vi "convertToHtml.vi"(8 "error in (no error)":errorcluster, 10 "HTML File Path":path, 11 "MS-Excel in":refnum<class "MS-Excel.lvclass">) -> (0 "error out":errorcluster, 3 "MS-Excel out":refnum<class "MS-Excel.lvclass">)   [LabVIEW 2017, in "LabVIEW NPOI.lvlib" / "MS-Excel.lvclass"]
uses:
  MS-Excel.lvclass
  MS-Excel.lvclass/MS-Excel.ctl
  C:/Program Files (x86)/National Instruments/LabVIEW 2017/vi.lib/BenjaminR/LabVIEW NPOI/lib/NPOI 2.1.1/NPOI.OOXML.dll
  Program Files (x86)/National Instruments/LabVIEW 2017/vi.lib/BenjaminR/LabVIEW NPOI/lib/NPOI 2.1.1/NPOI.OOXML.dll
  System.Xml
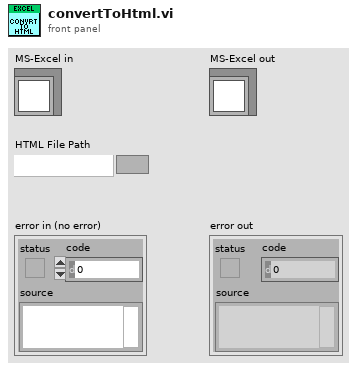
[diagram p1: front panel]
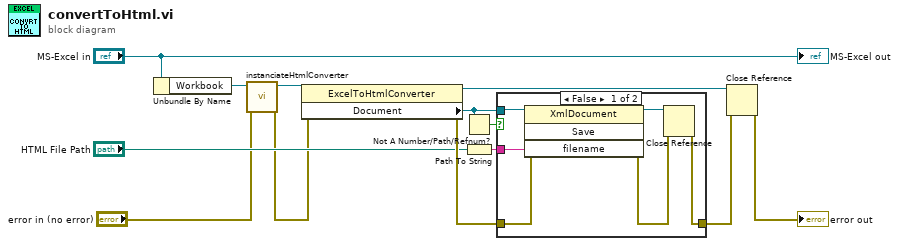
[diagram p0: block diagram]
diagram:
  n1 = Unbundle By Name("MS-Excel in") -> ("Workbook"=w3:refnum<k24>)
  n2 = call "instanciateHtmlConverter.vi"("error in (no error)"="error in (no error)", "workbook"=w3) -> ("error out"=w1:errorcluster, "ExcelToHtmlConverter"=w4:refnum<k24>)  [unwired: 8 in]
  n3 = property class="ExcelToHtmlConverter"(reference=w4, error in=w1) -> (reference out=w10:refnum<k24>, error out=w12:errorcluster, "Document"=w6:refnum<k24>)
  n4 = Not A Number/Path/Refnum?(number/path/refnum=w6) -> (NaN/Path/Refnum?=w7:bool)
  n5 = Path To String(path="HTML File Path") -> (string=w5:string)
  n6 = case shown="False" w7 {
    tunnel: w12 -> [w19 w20]
    tunnel: w5 -> [w18 _]
    tunnel: [w15 w20] -> w9
    tunnel: w6 -> [w14 _]
    frame False {
      n7 = invoke class="XmlDocument" method="Save"(reference=w14, error in=w19, "filename"=w18) -> (reference out=w17:refnum<k24>, error out=w16:errorcluster)  [unwired: 1 in, 2 out]
      n8 = Close Reference(reference=w17, error in (no error)=w16) -> (error out=w15:errorcluster)
    }
    frame True {
    }
  }
  n9 = Close Reference(reference=w10, error in (no error)=w9) -> (error out=→"error out":errorcluster)
  "MS-Excel out" <- "MS-Excel in"
